vi "Test Deposit Funds.vi"() -> ()   [LabVIEW 2026]
doc: "Caraya unit test for Deposit Funds.vi. Every case starts from its own fresh copy of the specification accounts file (Create Accounts Fixture.vi, written under Tests\\results), so the real ATM accounts.txt is never touched and the cases can run in parallel.\n\nCase 1: depositing 100 into 12345 (balance 550) returns the record with balance 650 AND the file holds 650 afterwards (read back with Get Account.vi).\nCase 2: depositing into the unknown account 99999 returns error 5003.\n\nThe error cluster carries the FIRST failure only. Read the JUnit report for all of them."
uses:
  <vilib>/addons/_JKI Toolkits/Caraya/classes/Test/Test.lvclass
  <vilib>/addons/_JKI Toolkits/Caraya/classes/Assert/Assert.lvclass
panel:
  out "error out":errorcluster
  in  "error in":errorcluster
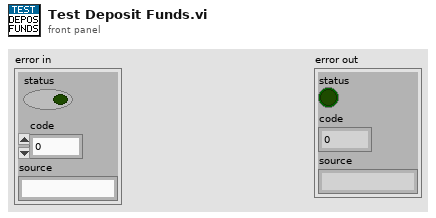
[diagram p1: front panel]
types:
  T1 = cluster{"Account Number":string, "First Name":string, "Last Name":string, "Balance":dbl}
  T2 = typedef "ATM Account.ctl" = cluster{"Account Number":string, "First Name":string, "Last Name":string, "Balance":dbl}
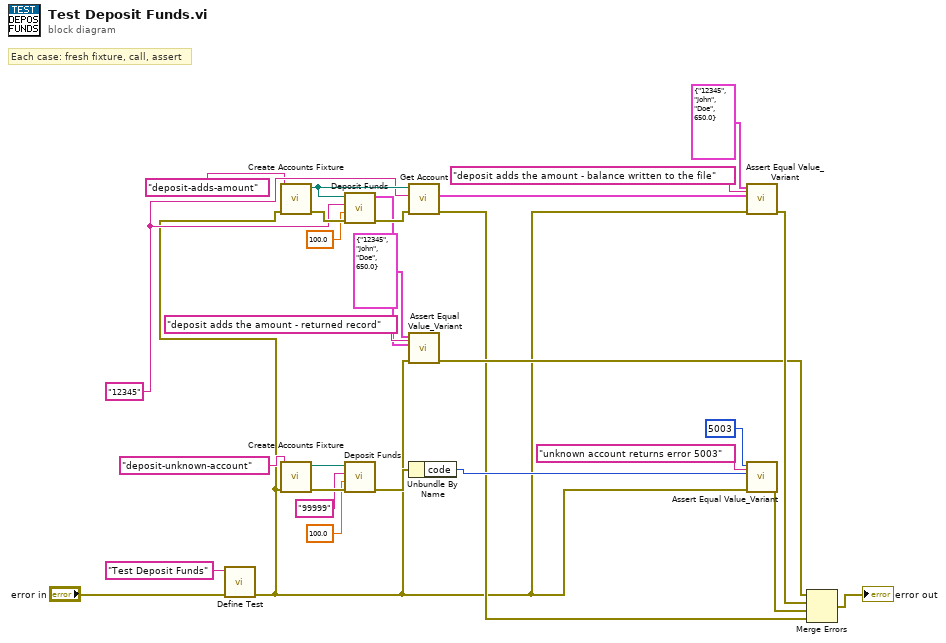
[diagram p0: block diagram]
diagram:
  w6 = "12345" ("Account Number")
  # "Each case: fresh fixture, call, assert"
  n1 = call <vilib>:"Define Test.vi"("error in (no error)"="error in", "Label (VI Title)"="Test Deposit Funds") -> ("error out"=w4:errorcluster)  [unwired: 8 in, 1 out]
  n2 = call "Create Accounts Fixture.vi"("error in"=w4, "Fixture Name"="deposit-adds-amount") -> ("error out"=w9:errorcluster, "Accounts File Path"=w8:path)  [unwired: 8 in]
  n3 = call "Create Accounts Fixture.vi"("error in"=w4, "Fixture Name"="deposit-unknown-account") -> ("error out"=w24:errorcluster, "Accounts File Path"=w23:path)  [unwired: 8 in]
  n4 = call "Deposit Funds.vi"("error in"=w9, "Amount"=100.0, "Account Number"=w6, "Accounts File Path"=w8) -> ("error out"=w11:errorcluster, "Account"=w10:T2)  [unwired: 6 in]
  n5 = call "Deposit Funds.vi"("error in"=w24, "Amount"=100.0, "Account Number"="99999", "Accounts File Path"=w23) -> ("error out"=w25:errorcluster)  [unwired: 6 in, 1 out]
  n6 = call "Get Account.vi"("error in"=w11, "Account Number"=w6, "Accounts File Path"=w8) -> ("error out"=w13:errorcluster, "Account"=w12:T2)  [unwired: 6 in, 1 out]
  n7 = call <vilib>:"Assert Equal Value_Variant.vi"("Label"="deposit adds the amount - returned record", "error in (no error)"=w4, "Actual"=w10, "Expected"=T1 {"Account Number"="12345", "First Name"="John", "Last Name"="Doe", "Balance"=650.0} ("expected 1")) -> ("error out"=w16:errorcluster)  [unwired: 6 in, 1 out]
  n8 = Unbundle By Name(w25) -> ("code"=w26:i32)
  n9 = call <vilib>:"Assert Equal Value_Variant.vi"("Label"="deposit adds the amount - balance written to the file", "error in (no error)"=w4, "Actual"=w12, "Expected"=T1 {"Account Number"="12345", "First Name"="John", "Last Name"="Doe", "Balance"=650.0} ("expected 2")) -> ("error out"=w19:errorcluster)  [unwired: 6 in, 1 out]
  n10 = call <vilib>:"Assert Equal Value_Variant.vi"("Label"="unknown account returns error 5003", "error in (no error)"=w4, "Actual"=w26, "Expected"=5003 ("expected 3")) -> ("error out"=w29:errorcluster)  [unwired: 6 in, 1 out]
  n11 = Merge Errors(w16, w19, w29, w13) -> (→"error out":errorcluster)
